vi "BNO055.vi"(8 "error in (no error)":errorcluster) -> (0 "error out":errorcluster, 3 "I2C Ref Out":T1)   [LabVIEW 2019]
uses:
  <vilib>/myRIO/Instrument Drivers/Onboard IO/I2C/typedefs/I2C Reference.ctl
  <vilib>/myRIO/Common/Instrument Driver Framework/Utilities/typedefs/myRIO Generic Hardware Reference.ctl
  <vilib>/myRIO/Common/Instrument Driver Framework/Utilities/typedefs/Hardware Version Enum.ctl
  <vilib>/myRIO/Common/Instrument Driver Framework/Utilities/typedefs/myRIO v1.0 Reference.ctl
  <vilib>/myRIO/Common/Instrument Driver Framework/Utilities/typedefs/Generic FPGA Reference.ctl
  <vilib>/myRIO/Common/Instrument Driver Framework/myRIO v1.0/I2C/typedefs/I2C Channels Enum.ctl
  <vilib>/myRIO/Instrument Drivers/Onboard IO/I2C/typedefs/I2C Configuration.ctl
  <vilib>/myRIO/Instrument Drivers/Onboard IO/I2C/typedefs/I2C Transfer Rate.ctl
  <vilib>/myRIO/Instrument Drivers/Onboard IO/I2C/typedefs/I2C User Configuration.ctl
  <vilib>/userDefined/High Color/nirio_resource_hc.ctl
  <vilib>/myRIO/Common/Instrument Driver Framework/myRIO v1.0/I2C/vis/myRIO v1.1 Open I2C.vi
  <vilib>/myRIO/Common/Instrument Driver Framework/Utilities/vis/Validate Channels.vi
  <vilib>/myRIO/Common/Instrument Driver Framework/myRIO v1.0/I2C/vis/myRIO v1.0 Reserve I2C.vi
  <vilib>/myRIO/Common/Instrument Driver Framework/myRIO v1.0/I2C/vis/myRIO v1.0 Build MUX Configuration I2C.vi
  <vilib>/myRIO/Common/Instrument Driver Framework/myRIO v1.0/Resource Manager/vis/myRIO v1.0 Reserve Channel List.vi
  <vilib>/myRIO/Common/Instrument Driver Framework/myRIO v1.0/Resource Manager/vis/myRIO v1.0 Create Configuration List.vi
  <vilib>/myRIO/Common/Instrument Driver Framework/myRIO v1.0/Resource Manager/vis/myRIO v1.0 Reserve Channel.vi
  <vilib>/myRIO/Common/Instrument Driver Framework/myRIO v1.0/Resource Manager/vis/myRIO v1.0 Unreserve Channel.vi
  <vilib>/myRIO/Common/Instrument Driver Framework/myRIO v1.0/Resource Manager/vis/myRIO v1.0 Build Mutex Name.vi
  <vilib>/Utility/VariantDataType/GetNumericInfo.vi
  <vilib>/Utility/error.llb/Error Cluster From Error Code.vi
  <vilib>/myRIO/Common/Instrument Driver Framework/myRIO v1.0/myRIO v1.1 Open.vi
  <vilib>/myRIO/Common/Instrument Driver Framework/Utilities/vis/IO Manager.vi
  <vilib>/myRIO/Common/Instrument Driver Framework/Utilities/vis/Configuration Manager.vi
  <vilib>/myRIO/Common/Instrument Driver Framework/myRIO v1.0/Resource Manager/vis/myRIO v1.0 Configure IO.vi
  <vilib>/myRIO/Common/Instrument Driver Framework/myRIO v1.0/myRIO v1.0 Close.vi
  <vilib>/myRIO/Common/Instrument Driver Framework/myRIO v1.0/I2C/vis/myRIO v1.0 Configure I2C.vi
  <vilib>/myRIO/Common/Instrument Driver Framework/myRIO v1.0/I2C/vis/myRIO v1.0 Write I2C.vi
  <vilib>/myRIO/Instrument Drivers/Onboard IO/I2C/vis/myRIO I2C Open.xnode
  <vilib>/myRIO/Instrument Drivers/Onboard IO/I2C/I2C.lvlib
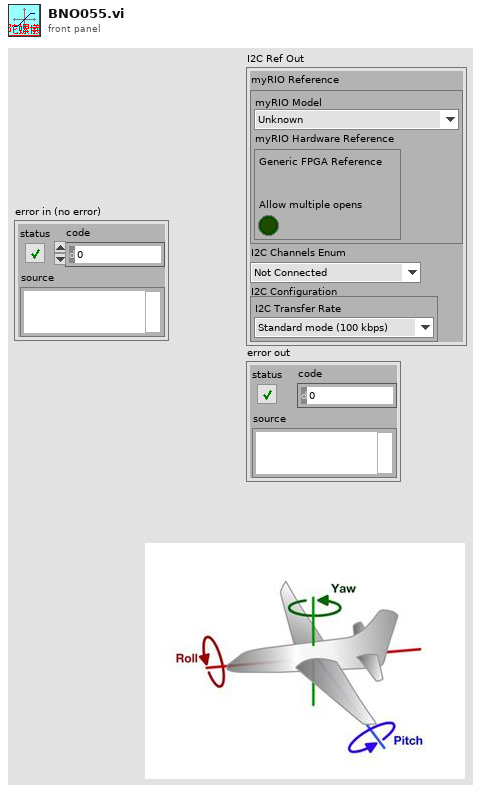
[diagram p1: front panel]
types:
  T1 = typedef "I2C.lvlib/I2C Reference.ctl" = cluster{"myRIO Reference":T2, "I2C Channels Enum":T6, "I2C Configuration":T7}
  T2 = typedef "myRIO Generic Hardware Reference.ctl" = cluster{"myRIO Model":T3, "myRIO Hardware Reference":T4}
  T3 = typedef "Hardware Version Enum.ctl" = enum16{"Unknown", "myRIO-1900", "myRIO-1950", "roboRIO", "NI ELVIS RIO CM", "ELVIS III"}
  T4 = typedef "myRIO v1.0 Reference.ctl" = cluster{"Generic FPGA Reference":T5, "Allow multiple opens":bool}
  T5 = typedef "Generic FPGA Reference.ctl" = refnum<k20>
  T6 = typedef "I2C Channels Enum.ctl" = enum16{"Not Connected", "A/I2C", "B/I2C", "I2C/I2C"}
  T7 = typedef "I2C.lvlib/I2C Configuration.ctl" = cluster{"I2C Transfer Rate":T8}
  T8 = typedef "I2C.lvlib/I2C Transfer Rate.ctl" = enum16{"Standard mode (100 kbps)", "Fast mode (400 kbps)"}
  T9 = typedef "I2C.lvlib/I2C User Configuration.ctl" = cluster{"I2C Transfer Rate":T8}
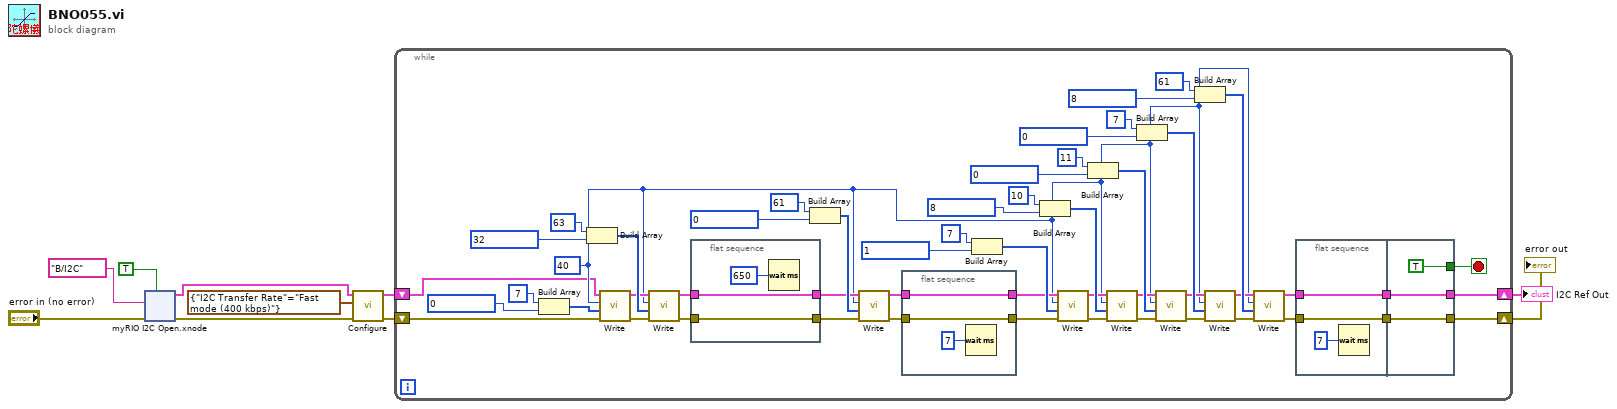
[diagram p0: block diagram]
diagram:
  n1 = xnode "myRIO I2C Open.xnode"("error in (no error)"="error in (no error)", "Allow multiple opens?"=TRUE, "Channel Name"=tag "B/I2C") -> ("error out"=w7:errorcluster, "I2C Ref Out"=w8:T1)
  n2 = call <vilib>:"Configure.vi"("error in (no error)"=w7, "I2C User Configuration"=T9 {"I2C Transfer Rate"=enum."Fast mode (400 kbps)"}, "I2C Ref In"=w8) -> ("error out"=w9:errorcluster, "I2C Ref Out"=w10:T1)  [unwired: 7 in]
  n3 = while {
    shift-right: [w22] -> w1
    shift-left: w9 -> [w15]
    shift-right: [w21] -> w2
    shift-left: w10 -> [w12]
    stop <- w18 stop-if-true
    w13 = 40
    n4 = Build Array(7, 0) -> (w14:i32[])
    n5 = Build Array(63, 32) -> (w61:i32[])
    n6 = call <vilib>:"Write.vi"("error in (no error)"=w15, "Bytes to Write"=w14, "Slave Address (7-bit)"=w13, "I2C Ref In"=w12) -> ("error out"=w17:errorcluster, "I2C Ref Out"=w16:T1)  [unwired: 6 in]
    n7 = call <vilib>:"Write.vi"("error in (no error)"=w17, "Bytes to Write"=w61, "Slave Address (7-bit)"=w13, "I2C Ref In"=w16) -> ("error out"=w52:errorcluster, "I2C Ref Out"=w54:T1)  [unwired: 6 in]
    n8 = flat-sequence {
      tunnel: [w73] -> w55
      tunnel: w54 -> [w73]
      tunnel: [w72] -> w53
      tunnel: w52 -> [w72]
      frame #0 {
        n9 = Wait (ms)(milliseconds to wait=u32 650) -> ()  [unwired: 1 out]
      }
    }
    n10 = Build Array(61, 0) -> (w56:i32[])
    n11 = call <vilib>:"Write.vi"("error in (no error)"=w53, "Bytes to Write"=w56, "Slave Address (7-bit)"=w13, "I2C Ref In"=w55) -> ("error out"=w50:errorcluster, "I2C Ref Out"=w51:T1)  [unwired: 6 in]
    n12 = flat-sequence {
      tunnel: [w70] -> w46
      tunnel: w51 -> [w70]
      tunnel: [w69] -> w45
      tunnel: w50 -> [w69]
      frame #0 {
        n13 = Wait (ms)(milliseconds to wait=u32 7) -> ()  [unwired: 1 out]
      }
    }
    n14 = Build Array(7, 1) -> (w49:i32[])
    n15 = Build Array(10, 8) -> (w42:i32[])
    n16 = call <vilib>:"Write.vi"("error in (no error)"=w45, "Bytes to Write"=w49, "Slave Address (7-bit)"=w13, "I2C Ref In"=w46) -> ("error out"=w40:errorcluster, "I2C Ref Out"=w41:T1)  [unwired: 6 in]
    n17 = Build Array(11, 0) -> (w39:i32[])
    n18 = call <vilib>:"Write.vi"("error in (no error)"=w40, "Bytes to Write"=w42, "Slave Address (7-bit)"=w13, "I2C Ref In"=w41) -> ("error out"=w35:errorcluster, "I2C Ref Out"=w36:T1)  [unwired: 6 in]
    n19 = Build Array(7, 0) -> (w32:i32[])
    n20 = call <vilib>:"Write.vi"("error in (no error)"=w35, "Bytes to Write"=w39, "Slave Address (7-bit)"=w13, "I2C Ref In"=w36) -> ("error out"=w30:errorcluster, "I2C Ref Out"=w31:T1)  [unwired: 6 in]
    n21 = Build Array(61, 8) -> (w29:i32[])
    n22 = call <vilib>:"Write.vi"("error in (no error)"=w30, "Bytes to Write"=w32, "Slave Address (7-bit)"=w13, "I2C Ref In"=w31) -> ("error out"=w26:errorcluster, "I2C Ref Out"=w25:T1)  [unwired: 6 in]
    n23 = call <vilib>:"Write.vi"("error in (no error)"=w26, "Bytes to Write"=w29, "Slave Address (7-bit)"=w13, "I2C Ref In"=w25) -> ("error out"=w23:errorcluster, "I2C Ref Out"=w24:T1)  [unwired: 6 in]
    n24 = flat-sequence {
      tunnel: w24 -> [w64]
      tunnel: w23 -> [w63]
      tunnel: [w64] -> w20
      tunnel: [w63] -> w19
      tunnel: [w67] -> w22
      tunnel: [w68] -> w21
      tunnel: w20 -> [w68]
      tunnel: w19 -> [w67]
      tunnel: [TRUE] -> w18
      frame #0 {
        n25 = Wait (ms)(milliseconds to wait=u32 7) -> ()  [unwired: 1 out]
      }
      frame #1 {
      }
    }
  }
  "I2C Ref Out" <- w2
  "error out" <- w1
